vi "Run_Many_VI.vi"(0 "Path":path[](array[path]), 11 "Error In":errorcluster) -> (4 "Refnum":refnum<vi>[](array[refnum]), 15 "Error Out":errorcluster)   [LabVIEW 2026, in "Core.lvlib"]
doc: "Opens multiple VIs from the specified paths and returns their corresponding VI references."
uses:
  Core.lvlib
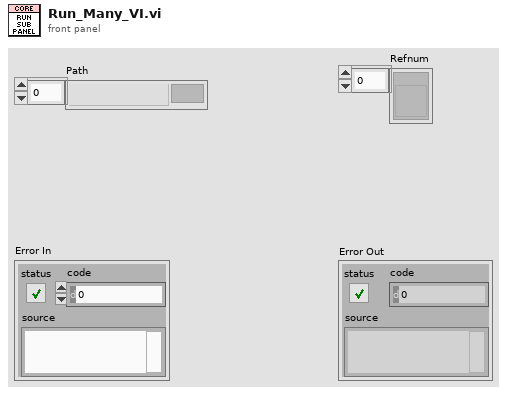
[diagram p1: front panel]
types:
  T1 = enum32{"Bad", "Idle", "Run top level", "Running"}
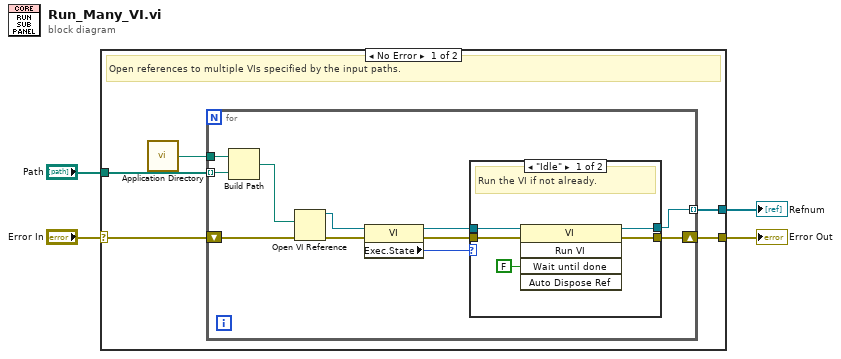
[diagram p0: block diagram]
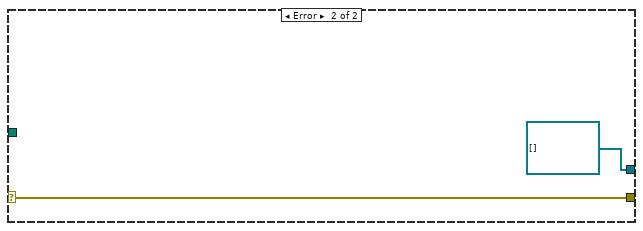
[diagram p3: hidden frame]
diagram:
  n1 = case shown="No Error" "Error In" {
    selector: "Error In" -> [w9 w29]
    tunnel: [w8 w29] -> w3
    tunnel: [w7 refnum<vi>[] []] -> w2
    tunnel: "Path" -> [w5 _]
    frame No Error {
      # "Open references to multiple VIs specified by the input paths."
      n2 = call <vilib>:"Application Directory.vi"() -> ("Application Directory"=w6:path)
      n3 = for {
        tunnel: [w12] -> w7 mode=indexing
        tunnel: w6 -> [w11]
        tunnel: w5 -> [w10] mode=indexing
        shift-right: [w13] -> w8
        shift-left: w9 -> [w17]
        n4 = Build Path(base path=w11, name or relative path=w10) -> (appended path=w14:path)
        n5 = Open VI Reference(vi path=w14, error in (no error)=w17) -> (vi reference=w15:refnum<vi>, error out=w16:errorcluster)  [unwired: 4 in]
        n6 = property class="VI"(reference=w15, error in=w16) -> (reference out=w20:refnum<vi>, error out=w19:errorcluster, "Exec.State"=w18:T1)
        n7 = case shown="\"Idle\"" w18 {
          tunnel: w19 -> [w25 w26]
          tunnel: w20 -> [w23 w27]
          tunnel: [w24 w26] -> w13
          tunnel: [w22 w27] -> w12
          frame "Idle" {
            # "Run the VI if not already."
            n8 = invoke class="VI" method="Run VI"(reference=w23, error in=w25, "Wait until done"=FALSE ("Wait Until Done")) -> (reference out=w22:refnum<vi>, error out=w24:errorcluster)  [unwired: 2 in, 3 out]
          }
          frame Default {
            # "Continue."
          }
        }
      }
    }
    frame Error {
    }
  }
  "Error Out" <- w3
  "Refnum" <- w2
